vi "PositionCtrl_TurnToAngle_Example.vi"() -> ()   [LabVIEW 2019]
uses:
  <vilib>/Rock Robotics/WPI/ThirdParty/JAS_Junk/TrajLib/MathUtil_Clamp.vi
  <vilib>/Rock Robotics/WPI/ThirdParty/JAS_Junk/TrajLib/Util_GetTime.vi
  <vilib>/Rock Robotics/WPI/ThirdParty/JAS_Junk/TrajLib/VI/MathUtil_RateOfChange.vi
  <vilib>/Rock Robotics/WPI/ThirdParty/JAS_Junk/TrajLib/VI/Util_GetTime_U32.vi
  <vilib>/Rock Robotics/WPI/ThirdParty/JAS_Junk/TrajLib/VI/Util_GetTime_U64.vi
  <vilib>/Rock Robotics/WPI/ThirdParty/JAS_Junk/TrajLib/Trajectory_Library.lvlib
panel:
  in  "Tab Control":T1(tab)
  out "Targets along the way":cluster{dbl, "PositionError":dbl, "modulus":dbl}(graph)
  in  "SP - Desired Angle\n (Deg)":dbl(slide) scale=-10.0..350.0
  out "PV - Current Angle\n (Deg)":dbl(slide) scale=-10.0..350.0
  out "Goal Chart":T2(graph)
  out "Motor Output":dbl format="%13.3f"
  out "Within Deadband":bool
  out "PositionError  (Deg)":dbl format="%13.2f"
  out "Velocity  (Deg/Sec)":dbl format="%13.2f"
  in  "Error Threshold\n(Deg)":dbl=25.0 format="%#_13g"
  in  "Error Tolerance\n(Deg)":dbl=0.5 format="%#_13g"
  in  "Output Deadband":dbl=0.08 format="%#_13g"
  in  "Output Threshold":dbl=1.0 format="%#_13g"
  in  "Kd":dbl format="%#_13g"
  out "Kp":dbl format="%#_13g"
  in  "Max Motor Output (+/-1)":dbl=1.0 format="%#_13g"
  in  "At Reference Count":i32=13
  # "BASIC TUNING PARAMETERS"
  # "Position Controller Tuning"
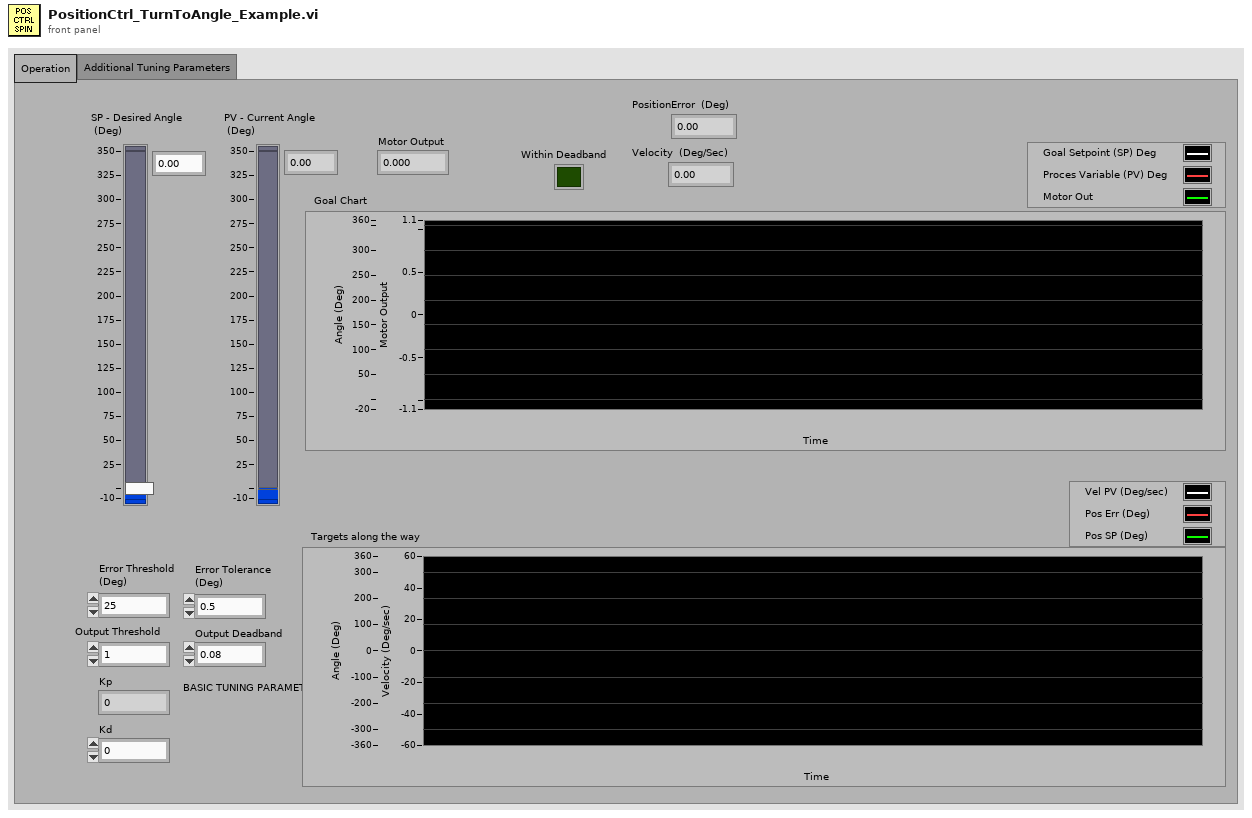
[diagram p1: front panel]
types:
  T1 = enum32{"Operation", "Additional Tuning Parameters"}
  T2 = cluster{"SP - Desired Position\n (Inch)":dbl, "upper limit":dbl, "upper limit":dbl}
  T3 = typedef "Trajectory_Library.lvlib/PosCtrl_Tuning_Type.ctl" = cluster{"Slope":dbl, "Offset":dbl, "Error Deadband":dbl, "At Reference Count":i32, "Negate Output":bool, "Max Allowd Position":dbl, "Min Allowd Position":dbl, "Kd":dbl}
  T4 = cluster{"SP - Desired Angle\n (Deg)":dbl, "modulus":dbl, "Output":dbl}
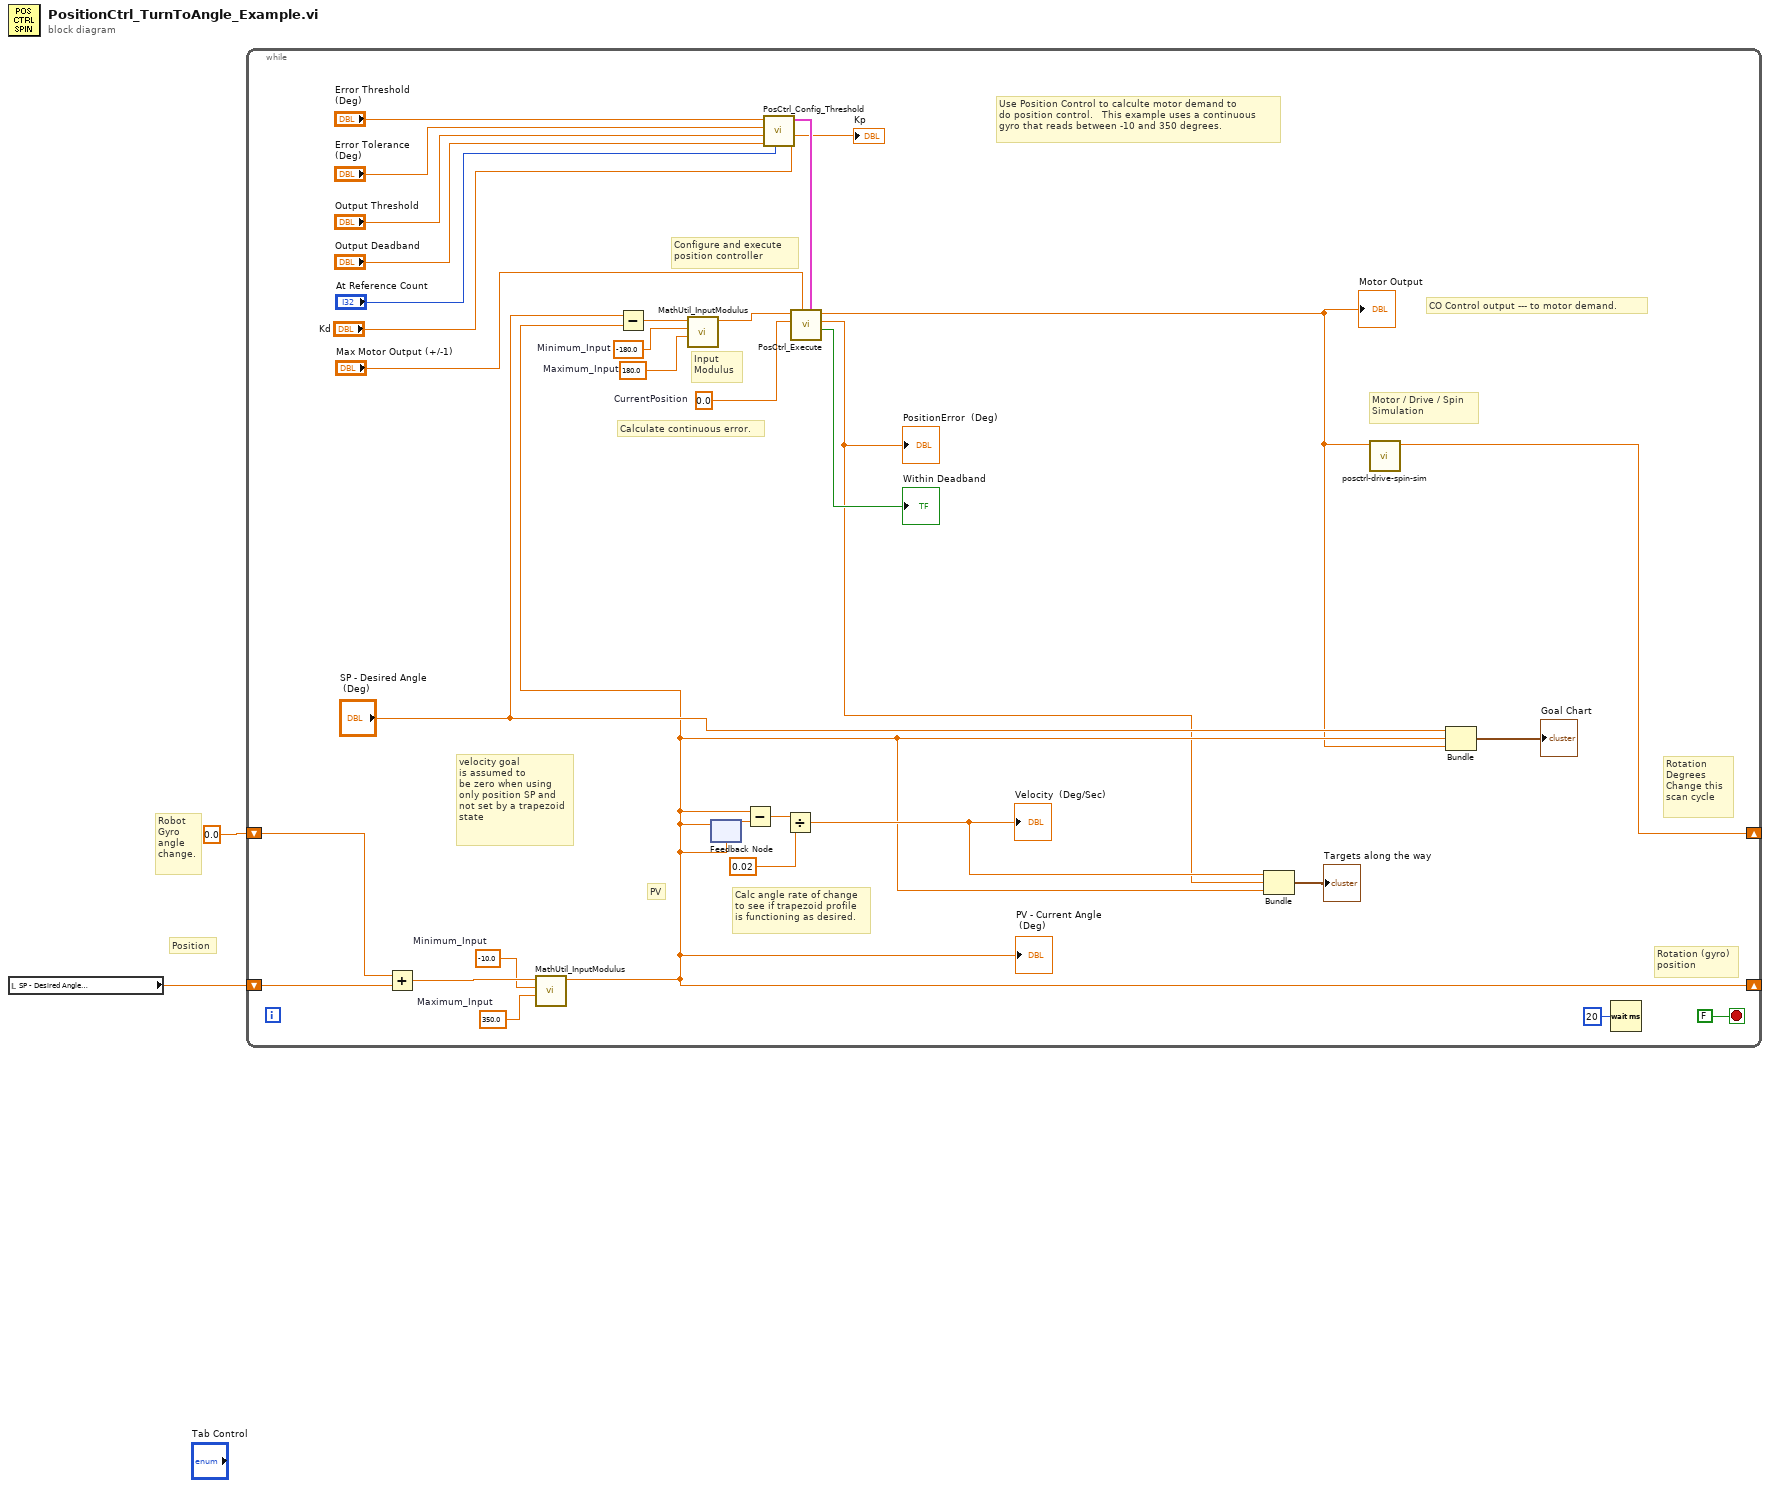
[diagram p0: block diagram]
diagram:
  # "Position"
  # "Robot\nGyro\nangle\nchange."
  n1 = local read "SP - Desired Angle\n (Deg)"() -> (w1:dbl)
  n2 = while {
    shift-right: [w15] -> _
    shift-left: w1 -> [w29]
    shift-right: [w23] -> _
    shift-left: 0.0 ("upper limit") -> [w24]
    stop <- FALSE stop-if-true
    w18 = -180.0  # Minimum_Input
    w20 = 180.0  # Maximum_Input
    w22 = 0.0  # CurrentPosition
    w25 = -10.0  # Minimum_Input
    w26 = 350.0  # Maximum_Input
    # "Calculate continuous error."
    # "Input\nModulus"
    # "Configure and execute \nposition controller"
    # "Use Position Control to calculte motor demand to\ndo position control.   This example uses a continuous\ngyro that reads between -10 and 350 degrees."
    # "Rotation (gyro)\nposition"
    # "Rotation\nDegrees \nChange this \nscan cycle"
    # "CO Control output --- to motor demand."
    # "Motor / Drive / Spin\nSimulation"
    # "PV"
    # "Calc angle rate of change\nto see if trapezoid profile\nis functioning as desired."
    # "velocity goal\nis assumed to \nbe zero when using\nonly position SP and\nnot set by a trapezoid\nstate"
    n3 = Add(x=w24, y=w29) -> (x+y=w27:dbl)
    n4 = call <vilib>:"MathUtil_InputModulus.vi"("Maximum_Input"=w26, "Minimum_Input"=w25, "Input"=w27) -> ("modulus"=w15:dbl)  [unwired: 8 in]
    "PV - Current Angle\n (Deg)" <- w15
    n5 = Subtract(x="SP - Desired Angle\n (Deg)", y=w15) -> (x-y=w17:dbl)
    n6 = call <vilib>:"MathUtil_InputModulus.vi"("Maximum_Input"=w20, "Minimum_Input"=w18, "Input"=w17) -> ("modulus"=w19:dbl)  [unwired: 8 in]
    n7 = feedback-in #1(w15) -> ()
    n8 = feedback #1(w15) -> (w33:dbl)
    n9 = Subtract(x=w15, y=w33) -> (x-y=w32:dbl)
    n10 = call <vilib>:"PosCtrl_Config_Threshold.vi"("Kd"="Kd", "At Reference Count"="At Reference Count", "Output Deadband"="Output Deadband", "Output Threshold"="Output Threshold", "ErrorDeadband"="Error Tolerance\n(Deg)", "ErrorThreshold"="Error Threshold\n(Deg)") -> ("Kp"=→"Kp":dbl, "PosCtrl_Config_Params"=w21:T3)  [unwired: 4 in]
    n11 = Divide(x=w32, y=0.02) -> (x/y=w28:dbl)
    "Velocity  (Deg/Sec)" <- w28
    n12 = call <vilib>:"PosCtrl_Execute.vi"("PosCtrl_Config_Params"=w21, "MaxOutput"="Max Motor Output (+/-1)", "CurrentPosition"=w22, "TargetPosition"=w19) -> ("OnTarget"=→"Within Deadband":bool, "PositionError"=w7:dbl, "Output"=w3:dbl)  [unwired: 5 in]
    "Motor Output" <- w3
    "PositionError  (Deg)" <- w7
    n13 = Bundle(w28, "PositionError"=w7, "modulus"=w15) -> (→"Targets along the way":cluster{dbl, "PositionError":dbl, "modulus":dbl})  [unwired: 1 in]
    n14 = call "posctrl-drive-spin-sim.vi"("Motor Demand"=w3) -> ("Rotation Change Deg"=w23:dbl)  [unwired: 10 in]
    n15 = Bundle("SP - Desired Angle\n (Deg)"="SP - Desired Angle\n (Deg)", "modulus"=w15, "Output"=w3) -> (→"Goal Chart":T4)  [unwired: 1 in]
    n16 = Wait (ms)(milliseconds to wait=u32 20) -> ()  [unwired: 1 out]
  }
